vi "BNO055 TEST.vi"() -> ()   [LabVIEW 2019]
panel:
  in  "stop":bool
  in  "error in (no error)":errorcluster
  out "Yaw":dbl
  out "Degrees":cluster{"Yaw":dbl, "Roll":dbl, "Pitch":dbl}
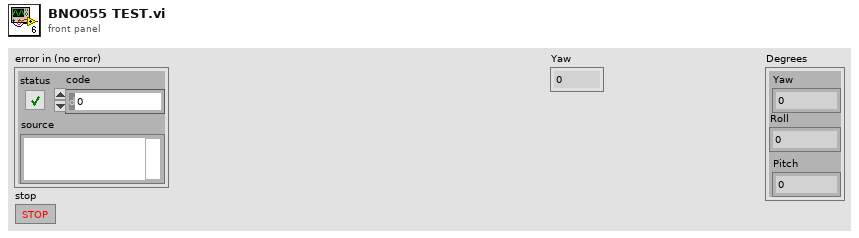
[diagram p1: front panel]
types:
  T1 = typedef "I2C.lvlib/I2C Reference.ctl" = cluster{"myRIO Reference":T2, "I2C Channels Enum":T6, "I2C Configuration":T7}
  T2 = typedef "myRIO Generic Hardware Reference.ctl" = cluster{"myRIO Model":T3, "myRIO Hardware Reference":T4}
  T3 = typedef "Hardware Version Enum.ctl" = enum16{"Unknown", "myRIO-1900", "myRIO-1950", "roboRIO", "NI ELVIS RIO CM", "ELVIS III"}
  T4 = typedef "myRIO v1.0 Reference.ctl" = cluster{"Generic FPGA Reference":T5, "Allow multiple opens":bool}
  T5 = typedef "Generic FPGA Reference.ctl" = refnum<k20>
  T6 = typedef "I2C Channels Enum.ctl" = enum16{"Not Connected", "A/I2C", "B/I2C", "I2C/I2C"}
  T7 = typedef "I2C.lvlib/I2C Configuration.ctl" = cluster{"I2C Transfer Rate":T8}
  T8 = typedef "I2C.lvlib/I2C Transfer Rate.ctl" = enum16{"Standard mode (100 kbps)", "Fast mode (400 kbps)"}
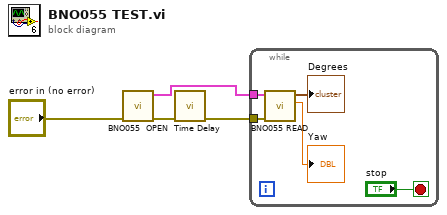
[diagram p0: block diagram]
diagram:
  n1 = call "BNO055  OPEN.vi"("error in (no error)"="error in (no error)") -> ("error out"=w3:errorcluster, "I2C Ref Out"=w1:T1)  [unwired: 9 in]
  n2 = call "Time Delay"("error in (no error)"=w3) -> ("error out"=w2:errorcluster)  [unwired: 10 in]
  n3 = while {
    tunnel: w2 -> [w7]
    tunnel: w1 -> [w6]
    stop <- "stop" stop-if-true
    n4 = call "BNO055 READ.vi"("error IN"=w7, "I2C Ref Out"=w6) -> ("Yaw"=→"Yaw":dbl, "Degrees"=→"Degrees":cluster{"Yaw":dbl, "Roll":dbl, "Pitch":dbl})  [unwired: 8 in]
  }
